vi "Read Publisher ID.vi"(11 "PublishRequest In":refnum<class "PublishRequest.lvclass">) -> (2 "Publisher ID":string)   [LabVIEW 2018, in "MVA Framework.lvlib" / "IMediator.lvlib" / "PublishRequest.lvclass"]
doc: "读取发布者ID"
uses:
  PublishRequest.lvclass
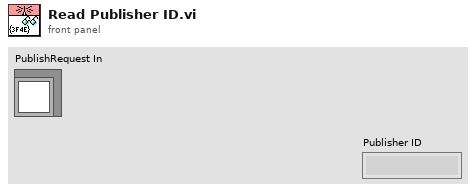
[diagram p1: front panel]
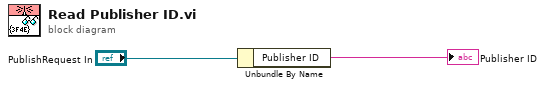
[diagram p0: block diagram]
diagram:
  n1 = Unbundle By Name("PublishRequest In") -> ("Publisher ID"=→"Publisher ID":string)
